vi "Day 12.vi"() -> ()   [LabVIEW 2021]
uses:
  <vilib>/Utility/file.llb/Read Delimited Spreadsheet (string).vi
panel:
  in  "Conditions":enum32{"Part 1", "Part 2"}(radio)
  out "Valid Paths":i32
  out "Valid Paths":string
  out "all rows":string[][](array[string])
  in  "Input File":T1(radio)
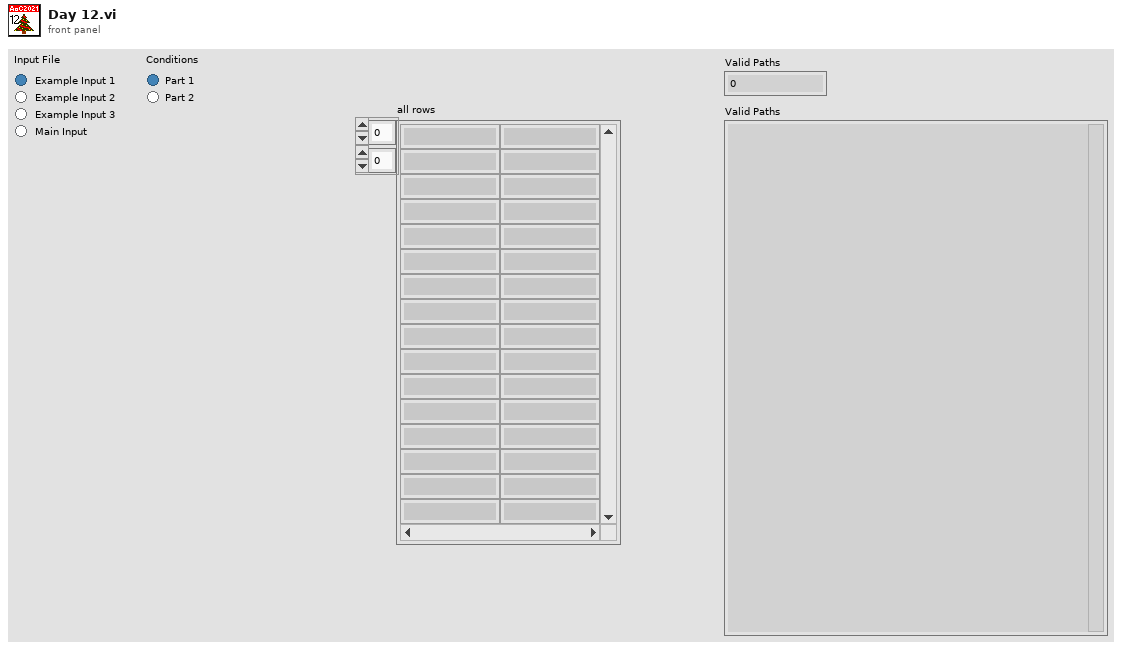
[diagram p1: front panel]
types:
  T1 = enum32{"Example Input 1", "Example Input 2", "Example Input 3", "Main Input"}
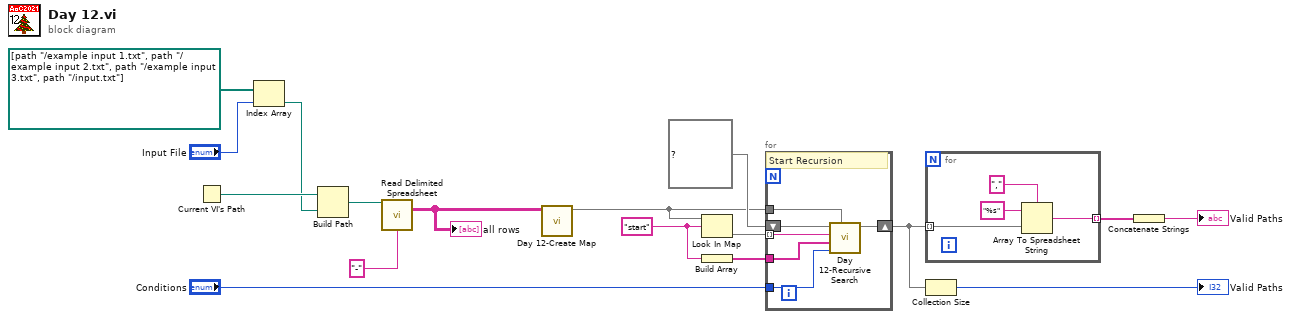
[diagram p0: block diagram]
diagram:
  w13 = "start" ("key")
  n1 = Current VI's Path() -> (path=w5:path)
  n2 = Index Array(array=path[] [path "../example input 1.txt", path "../example input 2.txt", path "../example input 3.txt", path "../input.txt"], index="Input File") -> (element=w3:path)
  n3 = Build Path(base path=w5, name or relative path=w3) -> (appended path=w4:path)
  n4 = call-poly <vilib>:"Read Delimited Spreadsheet.vi"("file path (dialog if empty)"=w4, "delimiter (\\t)"="-" ("delimiter (\\t)")) -> ("all rows"=w16:string[][])  [unwired: 8 in, 5 out]
  "all rows" <- w16
  n5 = call "Day 12-Create Map.vi"("Connections in"=w16) -> ("Map"=w1:map{string, set{string}})  [unwired: 10 in]
  n6 = Look In Map(map=w1, key=w13) -> (value=w15:set{string})  [unwired: 1 in, 1 out]
  n7 = Build Array(w13) -> (w14:string[])
  n8 = for {
    tunnel: w1 -> [w22]
    tunnel: w15 -> [w23] mode=indexing
    tunnel: w14 -> [w19]
    shift-right: [w20] -> w9
    shift-left: set{string[]} {} ("set in") -> [w21]
    tunnel: "Conditions" -> [w18]
    # "Start Recursion"
    n9 = call "Day 12-Recursive Search.vi"("Map"=w22, "Conditions"=w18, "Path in"=w19, "Next Cave"=w23, "Valid Paths in"=w21) -> ("Valid Paths out"=w20:set{string[]})  [unwired: 6 in]
  }
  n10 = for {
    tunnel: w9 -> [w24] mode=indexing
    tunnel: [w25] -> w11 mode=indexing
    n11 = Array To Spreadsheet String(delimiter (Tab)=",", array=w24, 3:"%s" ("format string")) -> (spreadsheet string=w25:string)
  }
  n12 = Collection Size(1:w9) -> (0:→"Valid Paths":i32)
  n13 = Concatenate Strings(w11) -> (→"Valid Paths":string)
